vi "Start If All Ready.vi"(8 "error in (no error)":errorcluster, 11 "Log Manager Module in":refnum<class "Log Manager Module.lvclass">) -> (0 "error out":errorcluster, 3 "Log Manager Module out":refnum<class "Log Manager Module.lvclass">)   [LabVIEW 2020, in "VolatusData.lvlib" / "Log Manager Module.lvclass"]
uses:
  Log Manager Module.lvclass
  C:/dev/lv20CE/relink/lv-volatus/Volatus/Module/Module.lvclass
  Log Manager Module.lvclass/Log Manager Module.ctl
  Logger State.ctl
  Logging State.ctl
  Volatus/MessageQ/MessageQ.lvclass/MessageQ.ctl
  Volatus/Module/Module.lvclass/Module.ctl
  Volatus/Module/Module.lvclass
  VolatusData.lvlib
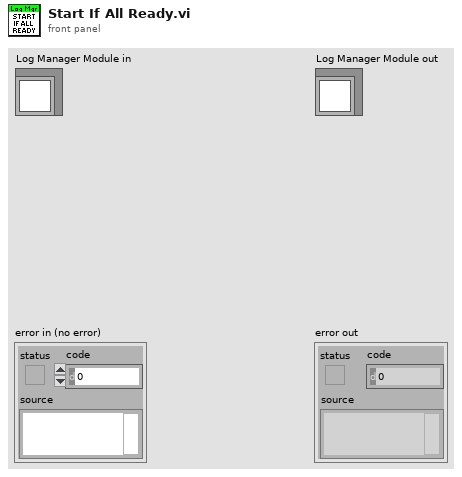
[diagram p1: front panel]
types:
  T1 = typedef "VolatusData.lvlib/Log Manager Module.lvclass/Group Info.ctl" = cluster{"Name":string, "Loggers":map{string, T2}}
  T2 = typedef "VolatusData.lvlib/Log Manager Module.lvclass/Logger.ctl" = cluster{"ID":string, "MsgQ":refnum<class "MessageQ.lvclass">, "State":T3, "Group":string}
  T3 = typedef "VolatusData.lvlib/Logger State.ctl" = enum16{"Unknown", "Idle", "Preparing", "Ready", "Logging", "Stopping"}
  T4 = typedef "VolatusData.lvlib/Logging State.ctl" = enum16{"Idle", "Starting", "Logging", "Stopping"}
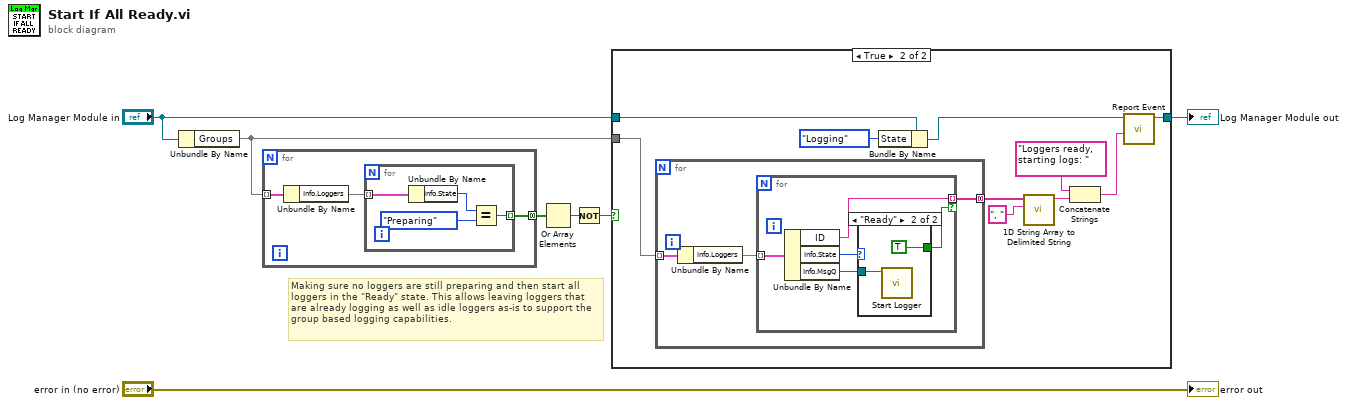
[diagram p0: block diagram]
diagram:
  # "Making sure no loggers are still preparing and then start all loggers in the \"Ready\" state. This allows leaving loggers that are already logging as well as idle loggers as-is to support the group based logging capabilities."
  n1 = Unbundle By Name("Log Manager Module in") -> ("Groups"=w5:map{string, T1})
  n2 = for {
    tunnel: w5 -> [w10] mode=indexing
    tunnel: [w9] -> w7 mode=concatenating
    n3 = Unbundle By Name(w10) -> ("Info.Loggers"=w8:map{string, T2})
    n4 = for {
      tunnel: [w12] -> w9 mode=indexing
      tunnel: w8 -> [w11] mode=indexing
      n5 = Unbundle By Name(w11) -> ("Info.State"=w14:T3)
      n6 = Equal?(x=w14, y=Logger_State."Preparing") -> (x = y?=w12:bool)
    }
  }
  n7 = Or Array Elements(Boolean array=w7) -> (logical OR=w6:bool)
  n8 = Not(x=w6) -> (.not. x?=w1:bool)
  n9 = case shown="True" w1 {
    tunnel: w5 -> [_ w25]
    tunnel: "Log Manager Module in" -> [w15 w16]
    tunnel: [w15 w18] -> w2
    frame False {
    }
    frame True {
      n10 = for {
        tunnel: w25 -> [w28] mode=indexing
        tunnel: [w26] -> w23 mode=concatenating
        n11 = Unbundle By Name(w28) -> ("Info.Loggers"=w27:map{string, T2})
        n12 = for {
          tunnel: w27 -> [w33] mode=indexing
          tunnel: [w30] -> w26 mode=indexing if=w29
          n13 = Unbundle By Name(w33) -> ("ID"=w30:string, "Info.State"=w31:T3, "Info.MsgQ"=w32:refnum<class "MessageQ.lvclass">)
          n14 = case shown="\"Ready\"" w31 {
            tunnel: w32 -> [_ w34]
            tunnel: [_ TRUE] -> w29
            frame Default {
            }
            frame "Ready" {
              n15 = call "Start Logger.vi"("MsgQ in"=w34) -> ()  [unwired: 9 in, 2 out]
            }
          }
        }
      }
      n16 = Bundle By Name(cluster=w16, "State"=Logging_State."Logging") -> (w17:refnum<class "Log Manager Module.lvclass">)
      n17 = call <vilib>:"1D String Array to Delimited String.vi"("delimiter"=", ", "string array"=w23) -> ("delimited string"=w21:string)  [unwired: 9 in]
      n18 = Concatenate Strings("Loggers ready, starting logs: " ("Message"), w21) -> (w19:string)
      n19 = call "Report Event.vi"("Message"=w19, "Module in"=w17) -> ("Module out"=w18:refnum<class "Log Manager Module.lvclass">)  [unwired: 8 in, 1 out]
    }
  }
  "Log Manager Module out" <- w2
  "error out" <- "error in (no error)"
